vi "_incrementHeadIndex.vi"(10 "NbElements":i32=1, 11 "VariantBuffer in":refnum<class "VariantBuffer.lvclass">) -> (3 "VariantBuffer out":refnum<class "VariantBuffer.lvclass">)   [LabVIEW 2013, in "CircularBuffer.lvlib" / "VariantBuffer.lvclass"]
uses:
  VariantBuffer.lvclass
  VariantBuffer.lvclass/VariantBuffer.ctl
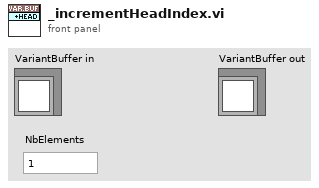
[diagram p1: front panel]
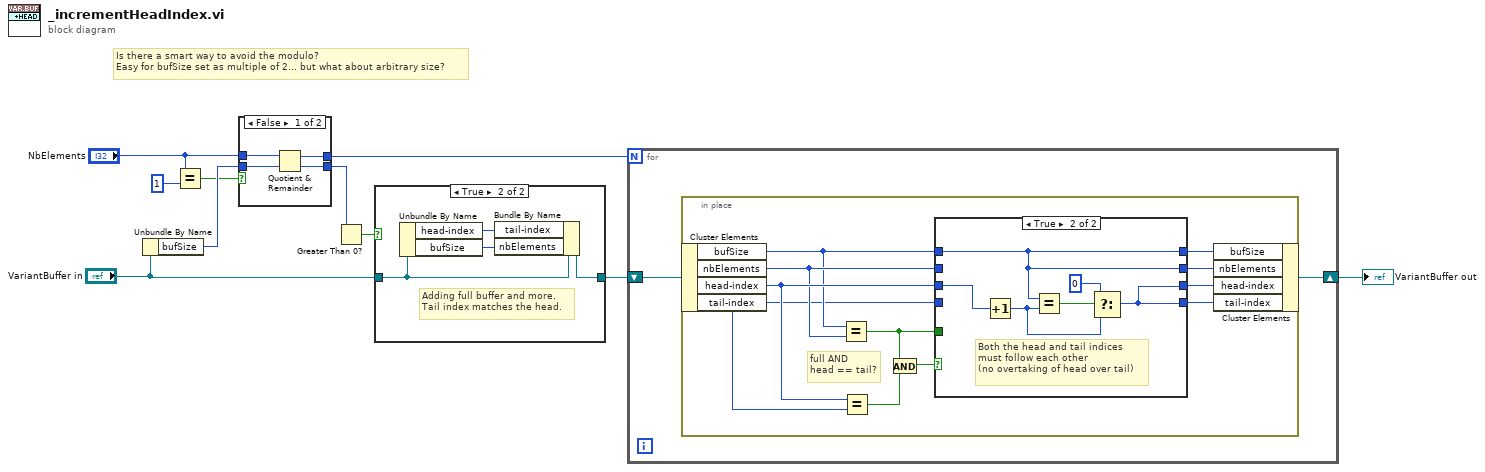
[diagram p0: block diagram]
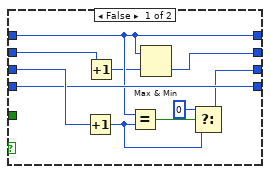
[diagram p2: hidden frame]
diagram:
  # "Is there a smart way to avoid the modulo?\nEasy for bufSize set as multiple of 2... but what about arbitrary size?"
  n1 = Unbundle By Name("VariantBuffer in") -> ("bufSize"=w9:i32)
  n2 = Equal?(x="NbElements", y=1) -> (x = y?=w5:bool)
  n3 = case shown="False" w5 {
    tunnel: w9 -> [w14 _]
    tunnel: [w13 w15] -> w8
    tunnel: [w12 _] -> w4
    tunnel: "NbElements" -> [w11 w15]
    frame False {
      n4 = Quotient & Remainder(x=w11, y=w14) -> (x-y*floor(x/y)=w13:i32, floor(x/y)=w12:i32)
    }
    frame True {
      # "1"
    }
  }
  n5 = Greater Than 0?(x=w4) -> (x > 0?=w3:bool)
  n6 = case shown="True" w3 {
    tunnel: [w16 w19] -> w1
    tunnel: "VariantBuffer in" -> [w16 w18]
    frame False {
    }
    frame True {
      # "Adding full buffer and more.\nTail index matches the head."
      n7 = Unbundle By Name(w18) -> ("head-index"=w17:i32, "bufSize"=w20:i32)
      n8 = Bundle By Name(cluster=w18, "tail-index"=w17, "nbElements"=w20) -> (w19:refnum<class "VariantBuffer.lvclass">)
    }
  }
  n9 = for {
    N: w8 -> [_]
    shift-right: [w22] -> w10
    shift-left: w1 -> [w21]
    n10 = in-place {
      # "full AND\nhead == tail?"
      n11 = in-place-cluster #1(w21) -> ("bufSize"=w28:i32, "nbElements"=w30:i32, "head-index"=w31:i32, "tail-index"=w24:i32)
      n12 = Equal?(x=w28, y=w30) -> (x = y?=w23:bool)
      n13 = Equal?(x=w31, y=w24) -> (x = y?=w29:bool)
      n14 = And(x=w23, y=w29) -> (x .and. y?=w25:bool)
      n15 = case shown="True" w25 {
        tunnel: [w34 w44] -> w33
        tunnel: [w35 w48] -> w32
        tunnel: w31 -> [w41 w49]
        tunnel: w30 -> [w38 _]
        tunnel: w28 -> [w37 w48]
        tunnel: [w37 w48] -> w27
        tunnel: [w40 w44] -> w26
        tunnel: w24 -> [w40 _]
        tunnel: w23 -> [_ _]
        frame False {
          n16 = Increment(x=w41) -> (x+1=w42:i32)
          n17 = Increment(x=w38) -> (x+1=w36:i32)
          n18 = Equal?(x=w37, y=w42) -> (x = y?=w39:bool)
          n19 = Max & Min(x=w37, y=w36) -> (min(x,y)=w35:i32)  [unwired: 1 out]
          n20 = Select(t=0, s=w39, f=w42) -> (s? t:f=w34:i32)
        }
        frame True {
          # "Both the head and tail indices\nmust follow each other \n(no overtaking of head over tail)"
          n21 = Increment(x=w49) -> (x+1=w45:i32)
          n22 = Equal?(x=w48, y=w45) -> (x = y?=w47:bool)
          n23 = Select(t=0, s=w47, f=w45) -> (s? t:f=w44:i32)
        }
      }
      n24 = in-place-cluster #1("bufSize"=w27, "nbElements"=w32, "head-index"=w33, "tail-index"=w26) -> (w22:refnum<class "VariantBuffer.lvclass">)
    }
  }
  "VariantBuffer out" <- w10
